vi "Price Return.vi"(5 "nervousness":dbl=1.0, 7 "shock":dbl, 8 "momentum":dbl, 9 "sector move":dbl, 10 "market move":dbl, 11 "stock":T1) -> (3 "return":dbl)   [LabVIEW 2020, in "Full Featured MCP Server.lvlib"]
doc: "The price model of one stock for one second. Returns the log return: the next price is price * exp(return), so a price can never fall to zero. return = drift + momentum + beta * market move + sector move + volatility * nervousness * noise + shock. The noise is a standard normal number; with the chance jumpiness it is four times as large."
uses:
  Full Featured MCP Server.lvlib
  Stock Entry.ctl
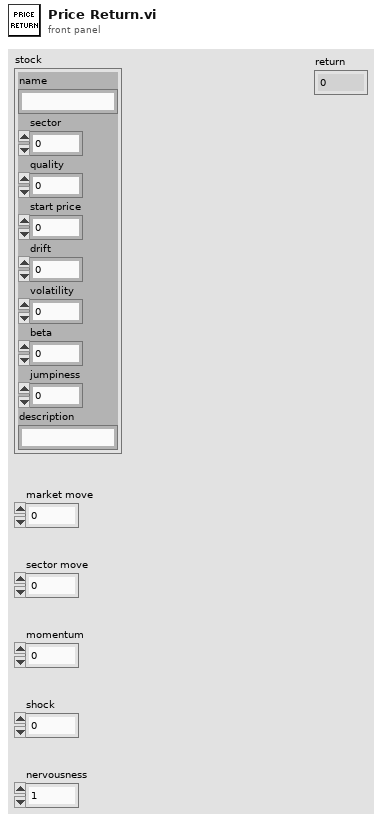
[diagram p1: front panel]
types:
  T1 = typedef "Full Featured MCP Server.lvlib/Stock Entry.ctl" = cluster{"name":string, "sector":i32, "quality":i32, "start price":dbl, "drift":dbl, "volatility":dbl, "beta":dbl, "jumpiness":dbl, "description":string}
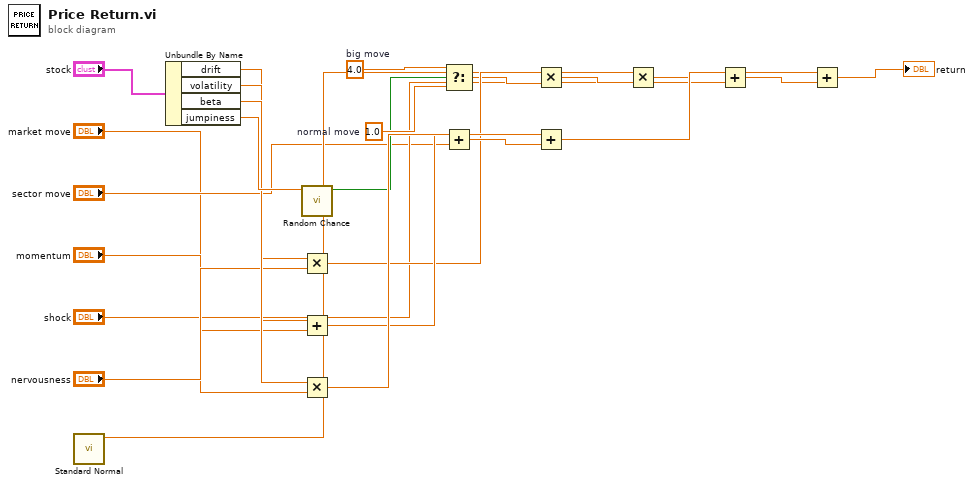
[diagram p0: block diagram]
diagram:
  w14 = 1.0  # normal move
  w13 = 4.0  # big move
  n1 = call "Standard Normal.vi"() -> ("number"=w12:dbl)  [unwired: 11 in]
  n2 = Unbundle By Name("stock") -> ("drift"=w7:dbl, "volatility"=w8:dbl, "beta"=w9:dbl, "jumpiness"=w10:dbl)
  n3 = call "Random Chance.vi"("probability"=w10) -> ("happened?"=w11:bool)  [unwired: 10 in]
  n4 = Multiply(x=w8, y="nervousness") -> (x*y=w17:dbl)
  n5 = Add(x=w7, y="momentum") -> (x+y=w19:dbl)
  n6 = Multiply(x=w9, y="market move") -> (x*y=w20:dbl)
  n7 = Select(t=w13, s=w11, f=w14) -> (s? t:f=w15:dbl)
  n8 = Add(x=w20, y="sector move") -> (x+y=w21:dbl)
  n9 = Multiply(x=w12, y=w15) -> (x*y=w16:dbl)
  n10 = Add(x=w19, y=w21) -> (x+y=w22:dbl)
  n11 = Multiply(x=w17, y=w16) -> (x*y=w18:dbl)
  n12 = Add(x=w18, y="shock") -> (x+y=w23:dbl)
  n13 = Add(x=w22, y=w23) -> (x+y=→"return":dbl)
